vi "lvmcp_addframe.vi"() -> ()   [LabVIEW 2026]
panel:
  out "reference out":refnum<vi>
  out "error out":errorcluster
  out "Add Frame":refnum<vi>
  in  "After? (T)":bool
  in  "Reference Frame Index":u32
  in  "reference":refnum<vi>
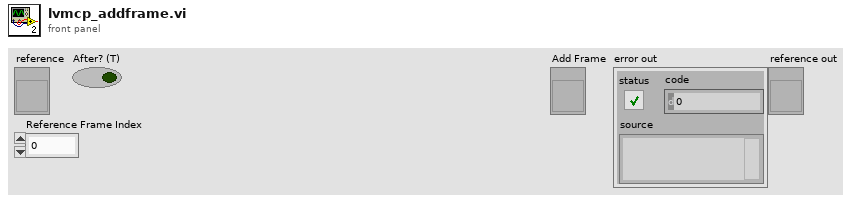
[diagram p1: front panel]
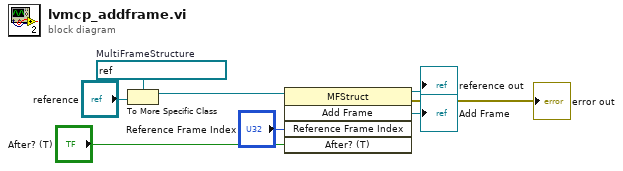
[diagram p0: block diagram]
diagram:
  w8 = refnum<vi> refnum  # MultiFrameStructure
  n1 = To More Specific Class(target class=w8, reference="reference") -> (specific class reference=w6:refnum<vi>)  [unwired: 1 in, 1 out]
  n2 = invoke class="MFStruct" method="Add Frame"(reference=w6, "Reference Frame Index"="Reference Frame Index", "After? (T)"="After? (T)") -> (reference out=→"reference out":refnum<vi>, error out=→"error out":errorcluster, "Add Frame"=→"Add Frame":refnum<vi>)  [unwired: 2 in, 2 out]
